vi "libssh2_channel_forward_listen_ex.vi"(7 "queue_maxsize":i32, 8 "error in (no error)":errorcluster, 9 "port in":i32, 10 "host":string, 11 "session":T2) -> (0 "error out":errorcluster, 1 "port out":i32, 3 "listener":T1)   [LabVIEW 2017, in "libssh2.lvlib"]
doc: "Create a listening channel for inbound TCP connections on a specific address and port on the SSH server. New connections are queued until accepted with <B>libssh2_channel_forward_accept</B>."
uses:
  libssh2.lvlib
  Session Refnum.ctl
  Listener Refnum.ctl
  Not A Session.vi
  <vilib>/Utility/error.llb/Error Cluster From Error Code.vi
  Global Settings.vi
  Read Session Refnum.vi
  <vilib>/Utility/semaphor.llb/Acquire Semaphore.vi
  <vilib>/Utility/semaphor.llb/Release Semaphore.vi
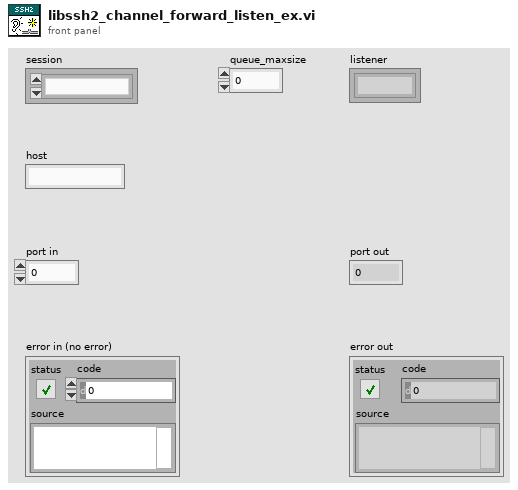
[diagram p1: front panel]
types:
  T1 = typedef "libssh2.lvlib/Listener Refnum.ctl" = refnum<k1>
  T2 = typedef "libssh2.lvlib/Session Refnum.ctl" = refnum<k1>
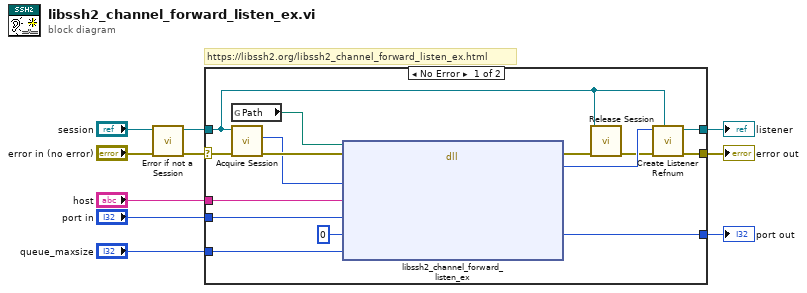
[diagram p0: block diagram]
diagram:
  # "https://libssh2.org/libssh2_channel_forward_listen_ex.html"
  n1 = call "Error if not a Session.vi"("error in (no error)"="error in (no error)", "session"="session") -> ("error out"=w3:errorcluster, "session out"=w1:T2)  [unwired: 8 in]
  n2 = case shown="No Error" w3 {
    selector: w3 -> [w14 w26]
    tunnel: "host" -> [w24 _]
    tunnel: "port in" -> [w23 _]
    tunnel: "queue_maxsize" -> [w22 _]
    tunnel: [w20 _] -> w7
    tunnel: w1 -> [w11 _]
    tunnel: [w17 w26] -> w6
    tunnel: [w15 _] -> w5
    frame No Error {
      n3 = global read "Global Settings.vi" "Path"() -> (w13:path)
      n4 = call "Acquire Session.vi"("error in (no error)"=w14, "session"=w11) -> ("error out"=w19:errorcluster, "LIBSSH2_SESSION*"=w18:u64)  [unwired: 7 in, 1 out]
      n5 = dll-call lib="?" fn="libssh2_channel_forward_listen_ex"(path in=w13, error in=w19, "session"=w18, "host"=w24, "port"=w23, "bound_port"=0, "queue_maxsize"=w22) -> (error out=w25:errorcluster, "return value"=w16:u64, "bound_port"=w20:i32)  [unwired: 5 in, 1 out]
      n6 = call "Release Session.vi"("error in (no error)"=w25, "session"=w11) -> ("error out"=w12:errorcluster)  [unwired: 9 in]
      n7 = call "Create Listener Refnum.vi"("session"=w11, "error in (no error)"=w12, "LIBSSH2_LISTENER*"=w16) -> ("error out"=w17:errorcluster, "listener"=w15:T1)  [unwired: 7 in]
    }
    frame Error {
    }
  }
  "error out" <- w6
  "port out" <- w7
  "listener" <- w5
